vi "FuncVI_Sub - VI - Convert LV data to CE data.vi"(5 "CE data type":T1=enum."DBL Number", 6 "error in":errorcluster, 8 "LV Type Descriptor":i16[](array[numeric]) format="%.0x", 9 "flattened data in":string) -> (0 "error out":errorcluster, 3 "flattened data out":string)   [LabVIEW 2021]
doc: "::: CalcExpress Toolkit :::\nCopyright (c) 2000-2026 Konstantin Shifershteyn. All rights reserved."
uses:
  cetypes.llb/CalcExpress Data Type.ctl
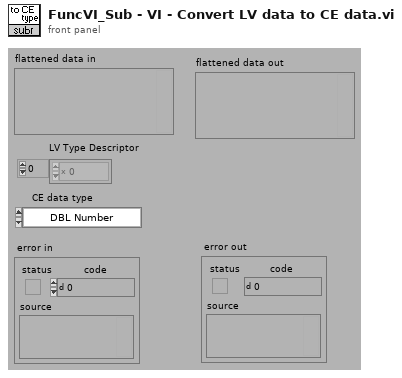
[diagram p1: front panel]
types:
  T1 = typedef "CalcExpress Data Type.ctl" = enum32{"String", "DBL Number", "identifier", "1D Array of DBL", "2D Array of DBL", "CDB Number", "1D Array of CDB", "2D Array of CDB", "1D Array of String", "2D Array of String", "Unknown data type"}
  T2 = enum16{"???", "int8", "int16", "int32", "float32", "float64", "float128", "complex32", "complex64", "complex128", "bool", "string", "path"}
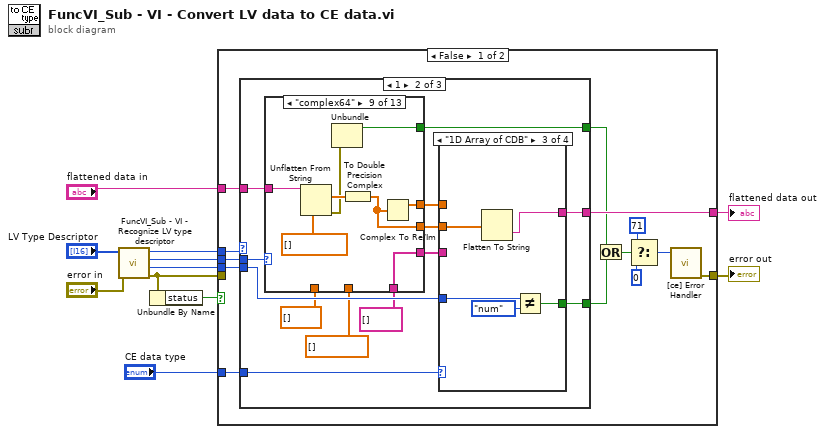
[diagram p0: block diagram]
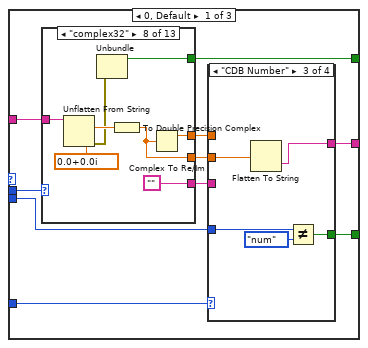
[diagram p2: hidden frame]
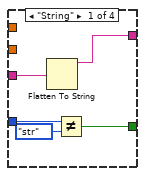
[diagram p3: hidden frame]
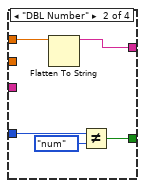
[diagram p4: hidden frame]
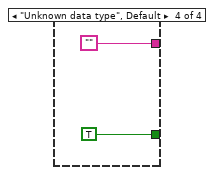
[diagram p5: hidden frame]
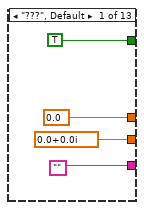
[diagram p6: hidden frame]
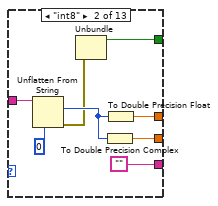
[diagram p7: hidden frame]
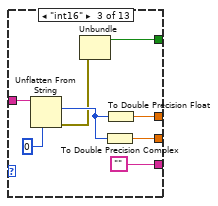
[diagram p8: hidden frame]
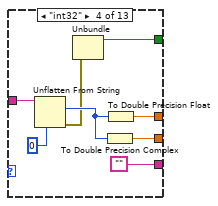
[diagram p9: hidden frame]
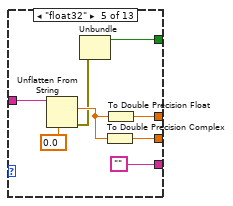
[diagram p10: hidden frame]
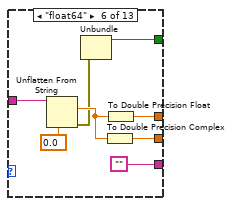
[diagram p11: hidden frame]
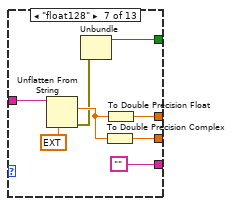
[diagram p12: hidden frame]
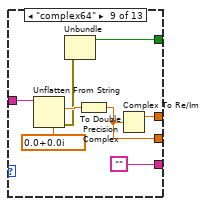
[diagram p13: hidden frame]
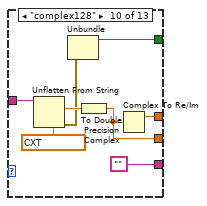
[diagram p14: hidden frame]
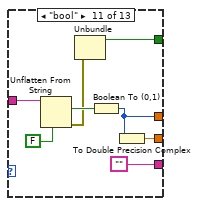
[diagram p15: hidden frame]
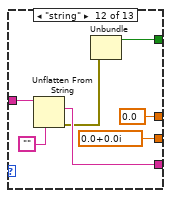
[diagram p16: hidden frame]
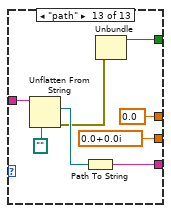
[diagram p17: hidden frame]
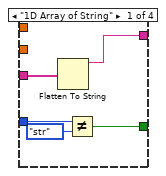
[diagram p18: hidden frame]
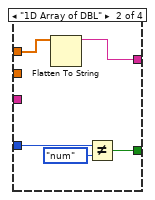
[diagram p19: hidden frame]
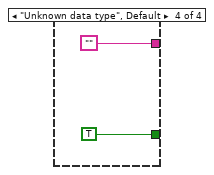
[diagram p20: hidden frame]
diagram:
  n1 = call "FuncVI_Sub - VI - Recognize LV type descriptor.vi"("error in"="error in", "Type Descriptor"="LV Type Descriptor") -> ("error out"=w2:errorcluster, "category"=w4:enum16{"num", "str"}, "representation"=w8:T2, "nDims"=w6:i32)  [unwired: 4 in]
  n2 = Unbundle By Name(w2) -> ("status"=w9:bool)
  n3 = case shown="False" w9 {
    tunnel: w8 -> [w24 _]
    tunnel: "flattened data in" -> [w23 w410]
    tunnel: w6 -> [w22 _]
    tunnel: "CE data type" -> [w21 _]
    tunnel: w4 -> [w20 _]
    tunnel: [w19 w410] -> w3
    tunnel: w2 -> [_ w409]
    tunnel: [w12 w409] -> w1
    frame False {
      n4 = case shown="1" w22 {
        tunnel: w24 -> [w34 w163 w292]
        tunnel: w23 -> [w33 w162 w291]
        tunnel: w21 -> [w31 w160 w289]
        tunnel: w20 -> [w28 w157 w286]
        tunnel: [w27 w156 w285] -> w16
        tunnel: [w26 w155 w284] -> w19
        tunnel: [w25 w151 w280] -> w15
        frame 0, Default {
          n5 = case shown="\"complex32\"" w34 {
            tunnel: w33 -> [_ w63 w71 w79 w87 w95 w103 w111 w119 w127 w135 w142 w150]
            tunnel: [0.0 w61 w69 w77 w85 w93 w101 w108 w116 w124 w130 0.0 0.0] -> w32
            tunnel: [cdb 0.0+0.0i w60 w68 w76 w84 w92 w100 w106 w114 w122 w131 cdb 0.0+0.0i cdb 0.0+0.0i] -> w30
            tunnel: ["" ("Empty String Constant") "" ("Empty String Constant") "" ("Empty String Constant") "" ("Empty String Constant") "" ("Empty String Constant") "" ("Empty String Constant") "" ("Empty String Constant") "" ("Empty String Constant") "" ("Empty String Constant") "" ("Empty String Constant") "" ("Empty String Constant") w140 w145] -> w29
            tunnel: [TRUE ("err") w57 w65 w73 w81 w89 w97 w105 w113 w121 w129 w137 w144] -> w25
            frame "???", Default {
            }
            frame "int8" {
              n6 = Unflatten From String(type=i8 0, binary string=w63) -> (value=w58:i8, error out=w56:errorcluster)  [unwired: 3 in, 1 out]
              n7 = Unbundle(w56) -> ("status"=w57:bool)  [unwired: 2 out]
              n8 = To Double Precision Complex(1:w58) -> (0:w60:cdb)
              n9 = To Double Precision Float(number=w58) -> (double precision float=w61:dbl)
            }
            frame "int16" {
              n10 = Unflatten From String(type=i16 0, binary string=w71) -> (value=w66:i16, error out=w64:errorcluster)  [unwired: 3 in, 1 out]
              n11 = Unbundle(w64) -> ("status"=w65:bool)  [unwired: 2 out]
              n12 = To Double Precision Complex(1:w66) -> (0:w68:cdb)
              n13 = To Double Precision Float(number=w66) -> (double precision float=w69:dbl)
            }
            frame "int32" {
              n14 = Unflatten From String(type=0, binary string=w79) -> (value=w74:i32, error out=w72:errorcluster)  [unwired: 3 in, 1 out]
              n15 = Unbundle(w72) -> ("status"=w73:bool)  [unwired: 2 out]
              n16 = To Double Precision Complex(1:w74) -> (0:w76:cdb)
              n17 = To Double Precision Float(number=w74) -> (double precision float=w77:dbl)
            }
            frame "float32" {
              n18 = Unflatten From String(type=sgl 0.0, binary string=w87) -> (value=w82:sgl, error out=w80:errorcluster)  [unwired: 3 in, 1 out]
              n19 = Unbundle(w80) -> ("status"=w81:bool)  [unwired: 2 out]
              n20 = To Double Precision Complex(1:w82) -> (0:w84:cdb)
              n21 = To Double Precision Float(number=w82) -> (double precision float=w85:dbl)
            }
            frame "float64" {
              n22 = Unflatten From String(type=0.0, binary string=w95) -> (value=w90:dbl, error out=w88:errorcluster)  [unwired: 3 in, 1 out]
              n23 = Unbundle(w88) -> ("status"=w89:bool)  [unwired: 2 out]
              n24 = To Double Precision Complex(1:w90) -> (0:w92:cdb)
              n25 = To Double Precision Float(number=w90) -> (double precision float=w93:dbl)
            }
            frame "float128" {
              n26 = Unflatten From String(type=ext 0.0, binary string=w103) -> (value=w98:ext, error out=w96:errorcluster)  [unwired: 3 in, 1 out]
              n27 = Unbundle(w96) -> ("status"=w97:bool)  [unwired: 2 out]
              n28 = To Double Precision Complex(1:w98) -> (0:w100:cdb)
              n29 = To Double Precision Float(number=w98) -> (double precision float=w101:dbl)
            }
            frame "complex32" {
              n30 = Unflatten From String(type=csg 0.0+0.0i, binary string=w111) -> (value=w107:csg, error out=w104:errorcluster)  [unwired: 3 in, 1 out]
              n31 = Unbundle(w104) -> ("status"=w105:bool)  [unwired: 2 out]
              n32 = To Double Precision Complex(1:w107) -> (0:w106:cdb)
              n33 = Complex To Re/Im(x + iy=w106) -> (x=w108:dbl)  [unwired: 1 out]
            }
            frame "complex64" {
              n34 = Unflatten From String(type=cdb 0.0+0.0i, binary string=w119) -> (value=w115:cdb, error out=w112:errorcluster)  [unwired: 3 in, 1 out]
              n35 = Unbundle(w112) -> ("status"=w113:bool)  [unwired: 2 out]
              n36 = To Double Precision Complex(1:w115) -> (0:w114:cdb)
              n37 = Complex To Re/Im(x + iy=w114) -> (x=w116:dbl)  [unwired: 1 out]
            }
            frame "complex128" {
              n38 = Unflatten From String(type=cxt 0.0+0.0i, binary string=w127) -> (value=w123:cxt, error out=w120:errorcluster)  [unwired: 3 in, 1 out]
              n39 = Unbundle(w120) -> ("status"=w121:bool)  [unwired: 2 out]
              n40 = To Double Precision Complex(1:w123) -> (0:w122:cdb)
              n41 = Complex To Re/Im(x + iy=w122) -> (x=w124:dbl)  [unwired: 1 out]
            }
            frame "bool" {
              n42 = Unflatten From String(type=FALSE, binary string=w135) -> (value=w132:bool, error out=w128:errorcluster)  [unwired: 3 in, 1 out]
              n43 = Unbundle(w128) -> ("status"=w129:bool)  [unwired: 2 out]
              n44 = Boolean To (0,1)(Boolean=w132) -> (0, 1=w130:i16)
              n45 = To Double Precision Complex(1:w130) -> (0:w131:cdb)
            }
            frame "string" {
              n46 = Unflatten From String(type="" ("Empty String Constant"), binary string=w142) -> (value=w140:string, error out=w136:errorcluster)  [unwired: 3 in, 1 out]
              n47 = Unbundle(w136) -> ("status"=w137:bool)  [unwired: 2 out]
            }
            frame "path" {
              n48 = Unflatten From String(type=path "" ("Empty Path Constant"), binary string=w150) -> (value=w148:path, error out=w143:errorcluster)  [unwired: 3 in, 1 out]
              n49 = Path To String(path=w148) -> (string=w145:string)
              n50 = Unbundle(w143) -> ("status"=w144:bool)  [unwired: 2 out]
            }
          }
          n51 = case shown="\"CDB Number\"" w31 {
            tunnel: w32 -> [_ w44 _ _]
            tunnel: w30 -> [_ _ w49 _]
            tunnel: w29 -> [w39 _ _ _]
            tunnel: w28 -> [w38 w43 w47 _]
            tunnel: [w36 w42 w46 TRUE] -> w27
            tunnel: [w35 w40 w45 "" ("Empty String Constant")] -> w26
            frame "String" {
              n52 = Flatten To String(anything=w39) -> (data string=w35:string)  [unwired: 3 in, 2 out]
              n53 = Not Equal?(x=w38, y=enum16{"num", "str"}."str") -> (x != y?=w36:bool)
            }
            frame "DBL Number" {
              n54 = Flatten To String(anything=w44) -> (data string=w40:string)  [unwired: 3 in, 2 out]
              n55 = Not Equal?(x=w43, y=enum16{"num", "str"}."num") -> (x != y?=w42:bool)
            }
            frame "CDB Number" {
              n56 = Flatten To String(anything=w49) -> (data string=w45:string)  [unwired: 3 in, 2 out]
              n57 = Not Equal?(x=w47, y=enum16{"num", "str"}."num") -> (x != y?=w46:bool)
            }
            frame "Unknown data type", Default {
            }
          }
        }
        frame 1 {
          n58 = case shown="\"complex64\"" w163 {
            tunnel: w162 -> [_ w192 w200 w208 w216 w224 w232 w240 w248 w256 w264 w271 w279]
            tunnel: [w182 w191 w199 w207 w215 w223 w231 w239 w247 w255 w261 w267 w274] -> w161
            tunnel: [w183 w190 w198 w206 w214 w222 w230 w237 w245 w253 w262 w268 w275] -> w159
            tunnel: [w184 w187 w196 w204 w212 w219 w227 w236 w244 w252 w260 w269 w276] -> w158
            tunnel: string[] [] -> [w184 w187 w196 w204 w212 w219 w227 w236 w244 w252 w260 _ _]
            tunnel: cdb[] [] -> [w183 _ _ _ _ _ _ _ _ _ _ w268 w275]
            tunnel: dbl[] [] -> [w182 _ _ _ _ _ _ _ _ _ _ w267 w274]
            tunnel: [TRUE ("err") w186 w194 w202 w210 w218 w226 w234 w242 w250 w258 w266 w273] -> w151
            frame "???", Default {
            }
            frame "int8" {
              n59 = Unflatten From String(type=i8[] [], binary string=w192) -> (value=w189:i8[], error out=w185:errorcluster)  [unwired: 3 in, 1 out]
              n60 = Unbundle(w185) -> ("status"=w186:bool)  [unwired: 2 out]
              n61 = To Double Precision Complex(1:w189) -> (0:w190:cdb[])
              n62 = To Double Precision Float(number=w189) -> (double precision float=w191:dbl[])
            }
            frame "int16" {
              n63 = Unflatten From String(type=i16[] [], binary string=w200) -> (value=w197:i16[], error out=w193:errorcluster)  [unwired: 3 in, 1 out]
              n64 = Unbundle(w193) -> ("status"=w194:bool)  [unwired: 2 out]
              n65 = To Double Precision Complex(1:w197) -> (0:w198:cdb[])
              n66 = To Double Precision Float(number=w197) -> (double precision float=w199:dbl[])
            }
            frame "int32" {
              n67 = Unflatten From String(type=i32[] [], binary string=w208) -> (value=w205:i32[], error out=w201:errorcluster)  [unwired: 3 in, 1 out]
              n68 = Unbundle(w201) -> ("status"=w202:bool)  [unwired: 2 out]
              n69 = To Double Precision Complex(1:w205) -> (0:w206:cdb[])
              n70 = To Double Precision Float(number=w205) -> (double precision float=w207:dbl[])
            }
            frame "float32" {
              n71 = Unflatten From String(type=sgl[] [], binary string=w216) -> (value=w213:sgl[], error out=w209:errorcluster)  [unwired: 3 in, 1 out]
              n72 = Unbundle(w209) -> ("status"=w210:bool)  [unwired: 2 out]
              n73 = To Double Precision Complex(1:w213) -> (0:w214:cdb[])
              n74 = To Double Precision Float(number=w213) -> (double precision float=w215:dbl[])
            }
            frame "float64" {
              n75 = Unflatten From String(type=dbl[] [], binary string=w224) -> (value=w221:dbl[], error out=w217:errorcluster)  [unwired: 3 in, 1 out]
              n76 = Unbundle(w217) -> ("status"=w218:bool)  [unwired: 2 out]
              n77 = To Double Precision Complex(1:w221) -> (0:w222:cdb[])
              n78 = To Double Precision Float(number=w221) -> (double precision float=w223:dbl[])
            }
            frame "float128" {
              n79 = Unflatten From String(type=ext[] [], binary string=w232) -> (value=w229:ext[], error out=w225:errorcluster)  [unwired: 3 in, 1 out]
              n80 = Unbundle(w225) -> ("status"=w226:bool)  [unwired: 2 out]
              n81 = To Double Precision Complex(1:w229) -> (0:w230:cdb[])
              n82 = To Double Precision Float(number=w229) -> (double precision float=w231:dbl[])
            }
            frame "complex32" {
              n83 = Unflatten From String(type=csg[] [], binary string=w240) -> (value=w238:csg[], error out=w233:errorcluster)  [unwired: 3 in, 1 out]
              n84 = Unbundle(w233) -> ("status"=w234:bool)  [unwired: 2 out]
              n85 = To Double Precision Complex(1:w238) -> (0:w237:cdb[])
              n86 = Complex To Re/Im(x + iy=w237) -> (x=w239:dbl[])  [unwired: 1 out]
            }
            frame "complex64" {
              n87 = Unflatten From String(type=cdb[] [], binary string=w248) -> (value=w246:cdb[], error out=w241:errorcluster)  [unwired: 3 in, 1 out]
              n88 = Unbundle(w241) -> ("status"=w242:bool)  [unwired: 2 out]
              n89 = To Double Precision Complex(1:w246) -> (0:w245:cdb[])
              n90 = Complex To Re/Im(x + iy=w245) -> (x=w247:dbl[])  [unwired: 1 out]
            }
            frame "complex128" {
              n91 = Unflatten From String(type=cxt[] [], binary string=w256) -> (value=w254:cxt[], error out=w249:errorcluster)  [unwired: 3 in, 1 out]
              n92 = Unbundle(w249) -> ("status"=w250:bool)  [unwired: 2 out]
              n93 = To Double Precision Complex(1:w254) -> (0:w253:cdb[])
              n94 = Complex To Re/Im(x + iy=w253) -> (x=w255:dbl[])  [unwired: 1 out]
            }
            frame "bool" {
              n95 = Unflatten From String(type=bool[] [], binary string=w264) -> (value=w263:bool[], error out=w257:errorcluster)  [unwired: 3 in, 1 out]
              n96 = Unbundle(w257) -> ("status"=w258:bool)  [unwired: 2 out]
              n97 = Boolean To (0,1)(Boolean=w263) -> (0, 1=w261:i16[])
              n98 = To Double Precision Complex(1:w261) -> (0:w262:cdb[])
            }
            frame "string" {
              n99 = Unflatten From String(type=string[] [], binary string=w271) -> (value=w269:string[], error out=w265:errorcluster)  [unwired: 3 in, 1 out]
              n100 = Unbundle(w265) -> ("status"=w266:bool)  [unwired: 2 out]
            }
            frame "path" {
              n101 = Unflatten From String(type=path[] [], binary string=w279) -> (value=w278:path[], error out=w272:errorcluster)  [unwired: 3 in, 1 out]
              n102 = Unbundle(w272) -> ("status"=w273:bool)  [unwired: 2 out]
              n103 = Path To String(path=w278) -> (string=w276:string[])
            }
          }
          n104 = case shown="\"1D Array of CDB\"" w160 {
            tunnel: w161 -> [_ w173 _ _]
            tunnel: w159 -> [_ _ w178 _]
            tunnel: w158 -> [w168 _ _ _]
            tunnel: w157 -> [w167 w172 w176 _]
            tunnel: [w165 w171 w175 TRUE] -> w156
            tunnel: [w164 w169 w174 "" ("Empty String Constant")] -> w155
            frame "1D Array of String" {
              n105 = Flatten To String(anything=w168) -> (data string=w164:string)  [unwired: 3 in, 2 out]
              n106 = Not Equal?(x=w167, y=enum16{"num", "str"}."str") -> (x != y?=w165:bool)
            }
            frame "1D Array of DBL" {
              n107 = Flatten To String(anything=w173) -> (data string=w169:string)  [unwired: 3 in, 2 out]
              n108 = Not Equal?(x=w172, y=enum16{"num", "str"}."num") -> (x != y?=w171:bool)
            }
            frame "1D Array of CDB" {
              n109 = Flatten To String(anything=w178) -> (data string=w174:string)  [unwired: 3 in, 2 out]
              n110 = Not Equal?(x=w176, y=enum16{"num", "str"}."num") -> (x != y?=w175:bool)
            }
            frame "Unknown data type", Default {
            }
          }
        }
        frame 2 {
          n111 = case shown="\"int8\"" w292 {
            tunnel: w291 -> [_ w321 w329 w337 w345 w353 w361 w369 w377 w385 w393 w400 w408]
            tunnel: [w311 w320 w328 w336 w344 w352 w360 w368 w376 w384 w390 w396 w403] -> w290
            tunnel: [w312 w319 w327 w335 w343 w351 w359 w366 w374 w382 w391 w397 w404] -> w288
            tunnel: [w313 w316 w325 w333 w341 w348 w356 w365 w373 w381 w389 w398 w405] -> w287
            tunnel: string[][] [] -> [w313 w316 w325 w333 w341 w348 w356 w365 w373 w381 w389 _ _]
            tunnel: cdb[][] [] -> [w312 _ _ _ _ _ _ _ _ _ _ w397 w404]
            tunnel: dbl[][] [] -> [w311 _ _ _ _ _ _ _ _ _ _ w396 w403]
            tunnel: [TRUE ("err") w315 w323 w331 w339 w347 w355 w363 w371 w379 w387 w395 w402] -> w280
            frame "???", Default {
            }
            frame "int8" {
              n112 = Unflatten From String(type=i8[][] [], binary string=w321) -> (value=w318:i8[][], error out=w314:errorcluster)  [unwired: 3 in, 1 out]
              n113 = Unbundle(w314) -> ("status"=w315:bool)  [unwired: 2 out]
              n114 = To Double Precision Complex(1:w318) -> (0:w319:cdb[][])
              n115 = To Double Precision Float(number=w318) -> (double precision float=w320:dbl[][])
            }
            frame "int16" {
              n116 = Unflatten From String(type=i16[][] [], binary string=w329) -> (value=w326:i16[][], error out=w322:errorcluster)  [unwired: 3 in, 1 out]
              n117 = Unbundle(w322) -> ("status"=w323:bool)  [unwired: 2 out]
              n118 = To Double Precision Complex(1:w326) -> (0:w327:cdb[][])
              n119 = To Double Precision Float(number=w326) -> (double precision float=w328:dbl[][])
            }
            frame "int32" {
              n120 = Unflatten From String(type=i32[][] [], binary string=w337) -> (value=w334:i32[][], error out=w330:errorcluster)  [unwired: 3 in, 1 out]
              n121 = Unbundle(w330) -> ("status"=w331:bool)  [unwired: 2 out]
              n122 = To Double Precision Complex(1:w334) -> (0:w335:cdb[][])
              n123 = To Double Precision Float(number=w334) -> (double precision float=w336:dbl[][])
            }
            frame "float32" {
              n124 = Unflatten From String(type=sgl[][] [], binary string=w345) -> (value=w342:sgl[][], error out=w338:errorcluster)  [unwired: 3 in, 1 out]
              n125 = Unbundle(w338) -> ("status"=w339:bool)  [unwired: 2 out]
              n126 = To Double Precision Complex(1:w342) -> (0:w343:cdb[][])
              n127 = To Double Precision Float(number=w342) -> (double precision float=w344:dbl[][])
            }
            frame "float64" {
              n128 = Unflatten From String(type=dbl[][] [], binary string=w353) -> (value=w350:dbl[][], error out=w346:errorcluster)  [unwired: 3 in, 1 out]
              n129 = Unbundle(w346) -> ("status"=w347:bool)  [unwired: 2 out]
              n130 = To Double Precision Complex(1:w350) -> (0:w351:cdb[][])
              n131 = To Double Precision Float(number=w350) -> (double precision float=w352:dbl[][])
            }
            frame "float128" {
              n132 = Unflatten From String(type=ext[][] [], binary string=w361) -> (value=w358:ext[][], error out=w354:errorcluster)  [unwired: 3 in, 1 out]
              n133 = Unbundle(w354) -> ("status"=w355:bool)  [unwired: 2 out]
              n134 = To Double Precision Complex(1:w358) -> (0:w359:cdb[][])
              n135 = To Double Precision Float(number=w358) -> (double precision float=w360:dbl[][])
            }
            frame "complex32" {
              n136 = Unflatten From String(type=csg[][] [], binary string=w369) -> (value=w367:csg[][], error out=w362:errorcluster)  [unwired: 3 in, 1 out]
              n137 = Unbundle(w362) -> ("status"=w363:bool)  [unwired: 2 out]
              n138 = To Double Precision Complex(1:w367) -> (0:w366:cdb[][])
              n139 = Complex To Re/Im(x + iy=w366) -> (x=w368:dbl[][])  [unwired: 1 out]
            }
            frame "complex64" {
              n140 = Unflatten From String(type=cdb[][] [], binary string=w377) -> (value=w375:cdb[][], error out=w370:errorcluster)  [unwired: 3 in, 1 out]
              n141 = Unbundle(w370) -> ("status"=w371:bool)  [unwired: 2 out]
              n142 = To Double Precision Complex(1:w375) -> (0:w374:cdb[][])
              n143 = Complex To Re/Im(x + iy=w374) -> (x=w376:dbl[][])  [unwired: 1 out]
            }
            frame "complex128" {
              n144 = Unflatten From String(type=cxt[][] [], binary string=w385) -> (value=w383:cxt[][], error out=w378:errorcluster)  [unwired: 3 in, 1 out]
              n145 = Unbundle(w378) -> ("status"=w379:bool)  [unwired: 2 out]
              n146 = To Double Precision Complex(1:w383) -> (0:w382:cdb[][])
              n147 = Complex To Re/Im(x + iy=w382) -> (x=w384:dbl[][])  [unwired: 1 out]
            }
            frame "bool" {
              n148 = Unflatten From String(type=bool[][] [], binary string=w393) -> (value=w392:bool[][], error out=w386:errorcluster)  [unwired: 3 in, 1 out]
              n149 = Unbundle(w386) -> ("status"=w387:bool)  [unwired: 2 out]
              n150 = Boolean To (0,1)(Boolean=w392) -> (0, 1=w390:i16[][])
              n151 = To Double Precision Complex(1:w390) -> (0:w391:cdb[][])
            }
            frame "string" {
              n152 = Unflatten From String(type=string[][] [], binary string=w400) -> (value=w398:string[][], error out=w394:errorcluster)  [unwired: 3 in, 1 out]
              n153 = Unbundle(w394) -> ("status"=w395:bool)  [unwired: 2 out]
            }
            frame "path" {
              n154 = Unflatten From String(type=path[][] [], binary string=w408) -> (value=w407:path[][], error out=w401:errorcluster)  [unwired: 3 in, 1 out]
              n155 = Path To String(path=w407) -> (string=w405:string[][])
              n156 = Unbundle(w401) -> ("status"=w402:bool)  [unwired: 2 out]
            }
          }
          n157 = case shown="\"2D Array of DBL\"" w289 {
            tunnel: w290 -> [_ w302 _ _]
            tunnel: w288 -> [_ _ w307 _]
            tunnel: w287 -> [w297 _ _ _]
            tunnel: w286 -> [w296 w301 w305 _]
            tunnel: [w294 w300 w304 TRUE] -> w285
            tunnel: [w293 w298 w303 "" ("Empty String Constant")] -> w284
            frame "2D Array of String" {
              n158 = Flatten To String(anything=w297) -> (data string=w293:string)  [unwired: 3 in, 2 out]
              n159 = Not Equal?(x=w296, y=enum16{"num", "str"}."str") -> (x != y?=w294:bool)
            }
            frame "2D Array of DBL" {
              n160 = Flatten To String(anything=w302) -> (data string=w298:string)  [unwired: 3 in, 2 out]
              n161 = Not Equal?(x=w301, y=enum16{"num", "str"}."num") -> (x != y?=w300:bool)
            }
            frame "2D Array of CDB" {
              n162 = Flatten To String(anything=w307) -> (data string=w303:string)  [unwired: 3 in, 2 out]
              n163 = Not Equal?(x=w305, y=enum16{"num", "str"}."num") -> (x != y?=w304:bool)
            }
            frame "Unknown data type", Default {
            }
          }
        }
      }
      n164 = Or(x=w15, y=w16) -> (x .or. y?=w14:bool)
      n165 = Select(t=71, s=w14, f=0) -> (s? t:f=w13:i32)
      n166 = call "[ce] Error Handler.vi"("error code"=w13) -> ("error out"=w12:errorcluster)  [unwired: 9 in, 1 out]
    }
    frame True {
    }
  }
  "flattened data out" <- w3
  "error out" <- w1
